vi "Submodule EOL UI.vi"() -> ()   [LabVIEW 2025, in "Submodule EOL.lvlib" / "Submodule EOL.lvclass"]
doc: "Copyright 2017 National Instruments Corporation\n\nLicensed under the Apache License, Version 2.0 (the \"License\"); you may not use this file except in compliance with the License. You may obtain a copy of the License at http://www.apache.org/licenses/LICENSE-2.0\nUnless required by applicable law or agreed to in writing, software distributed under the License is distributed on an \"AS IS\" BASIS, WITHOUT WARRANTIES OR CONDITIONS OF ANY KIND, either express or implied. See the License for the specific language governing permissions and limitations under the License."
uses:
  Submodule EOL.lvclass
  Users/Public/Documents/Sandia National Labs/TSS Plugin/CEF.lvlibp/Node/mainQref.ctl
  Users/Public/Documents/Sandia National Labs/TSS Plugin/CEF.lvlibp/Node/UserEventRef.ctl
  Submodule EOL configuration/Setting.ctl
  Submodule EOL configuration/PLC.ctl
  Users/Public/Documents/Sandia National Labs/TSS Plugin/CEF.lvlibp/Node/NodeRef.ctl
  Users/Public/Documents/Sandia National Labs/TSS Plugin/CEF.lvlibp/Node/CEF_Node.lvclass
  Submodule EOL configuration/Instrumnet.ctl
  Submodule EOL.lvclass/Submodule EOL.ctl
  Submodule EOL configuration/Submodule EOL configuration.lvclass/Submodule EOL configuration.ctl
  <vilib>/Utility/miscctls.llb/LVPositionTypeDef.ctl
  Submodule EOL configuration/Read Setting.vi
  Submodule EOL configuration/Read PLC.vi
  Submodule EOL configuration/Read Instrument.vi
  Submodule EOL configuration/Write Setting.vi
  Submodule EOL configuration/Write PLC.vi
  Submodule EOL configuration/Write Instrument.vi
  Submodule EOL configuration/Submodule EOL configuration.lvclass
panel:
  in  "Instrument":T1
  in  "node ref":T2
  in  "PLC":T3={"PLC Folder Names"=[["Station0_Rx", "OP50A_TesterRxSignals"], ["Station0_Tx", "OP50A_TesterTxSignals"], ["Station1_Rx", "OP50B_TesterRxSignals"], ["Station1_Tx", "OP50B_TesterTxSignals"], ["Station2_Rx", "OP60A_TesterRxSignals"], ["Station2_Tx", "OP60A_TesterTxSignals"], ["Station3_Rx", "OP60B_TesterRxSignals"], ["Station3_Tx", "OP60B_TesterTxSignals"], ["Station4_Rx", "OP70A_TesterRxSignals"], ["Station4_Tx", "OP70A_TesterTxSignals"], ["Station5_Rx", "OP70B_TesterRxSignals"], ["Station5_Tx", "OP70B_TesterTxSignals"]], "PLC URL"="opc.tcp://localhost:49580 ", "Ignition Folder Names"=[["Ignition0_Rx", "[Submodule_EOL]/StaA/TesterRx"], ["Ignition0_Tx", "[Submodule_EOL]/StaA/TesterTx"], ["Ignition1_Rx", "[Submodule_EOL]/StaB/TesterRx"], ["Ignition1_Tx", "[Submodule_EOL]/StaB/TesterTx"], ["Ignition2_Rx", "[Submodule_EOL]/StaC/TesterRx"], ["Ignition2_Tx", "[Submodule_EOL]/StaC/TesterTx"], ["Ignition3_Rx", "[Submodule_EOL]/StaD/TesterRx"], ["Ignition3_Tx", "[Submodule_EOL]/StaD/TesterTx"], ["Ignition4_Rx", "[Submodule_EOL]/StaE/TesterRx"], ["Ignition4_Tx", "[Submodule_EOL]/StaE/TesterTx"], ["Ignition5_Rx", "[Submodule_EOL]/StaF/TesterRx"], ["Ignition5_Tx", "[Submodule_EOL]/StaF/TesterTx"]], "Ignition URL"="opc.tcp://10.64.0.22:62541/discovery", "Test Name"="Battery Submodule EOL"}
  in  "Segmented":enum32{"PLC", "Setting", "Instrument"}(radio)
  in  "Setting":T4={"Local Database"="", "Connect OPC Trial"=0, "Timeout Connect OPC"=0.0, "AbstractUUT Path"="", "PreUUT Path"="", "Test Path"="", "PostUUT Path"="Battery Submodule End of Line"} {"Timeout Connect OPC" format="%#_f"}
  in  "user event":T5
  in  "main queue":T6
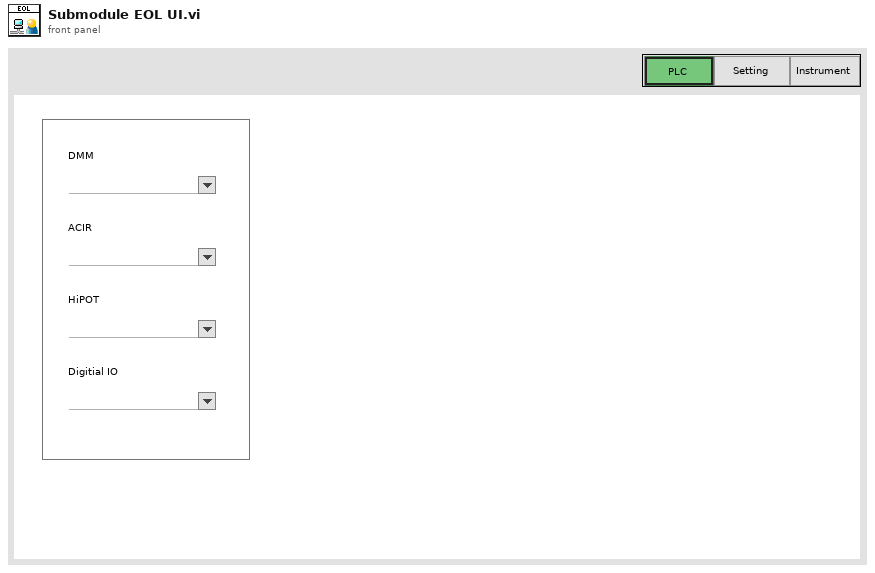
[diagram p1: front panel]
types:
  T1 = typedef "Submodule EOL.lvlib/Submodule EOL configuration.lvclass/Instrumnet.ctl" = cluster{"Digitial IO":string, "HiPOT":string, "ACIR":string, "DMM":string}
  T2 = typedef "CEF.lvlibp/CEF_Node.lvclass/NodeRef.ctl" = refnum<data-value>
  T3 = typedef "Submodule EOL.lvlib/Submodule EOL configuration.lvclass/PLC.ctl" = cluster{"PLC Folder Names":string[][], "PLC URL":string, "Ignition Folder Names":string[][], "Ignition URL":string, "Test Name":string}
  T4 = typedef "Submodule EOL.lvlib/Submodule EOL configuration.lvclass/Setting.ctl" = cluster{"Local Database":string, "Connect OPC Trial":u32, "Timeout Connect OPC":dbl, "AbstractUUT Path":string, "PreUUT Path":string, "Test Path":string, "PostUUT Path":string}
  T5 = typedef "CEF.lvlibp/CEF_Node.lvclass/UserEventRef.ctl" = refnum<user-event>
  T6 = typedef "CEF.lvlibp/CEF_Node.lvclass/mainQref.ctl" = refnum<queue>
  T7 = typedef "LVPositionTypeDef.ctl" = cluster{"Left":i32, "Top":i32}
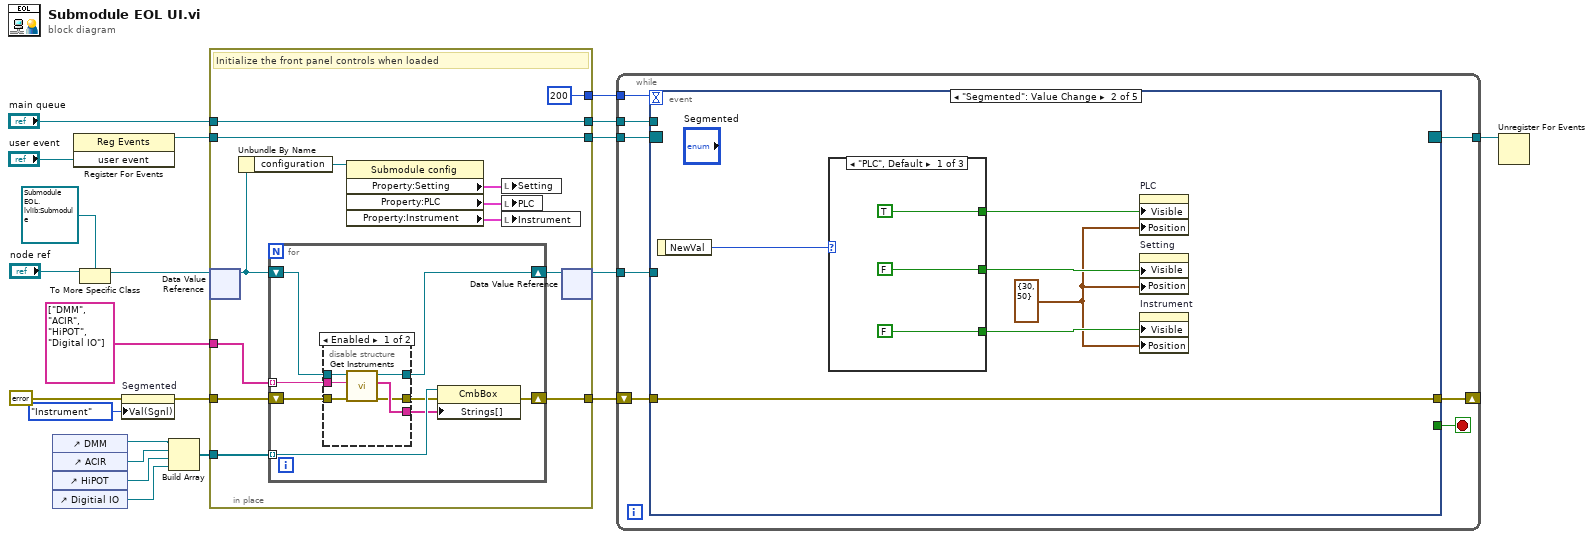
[diagram p0: block diagram]
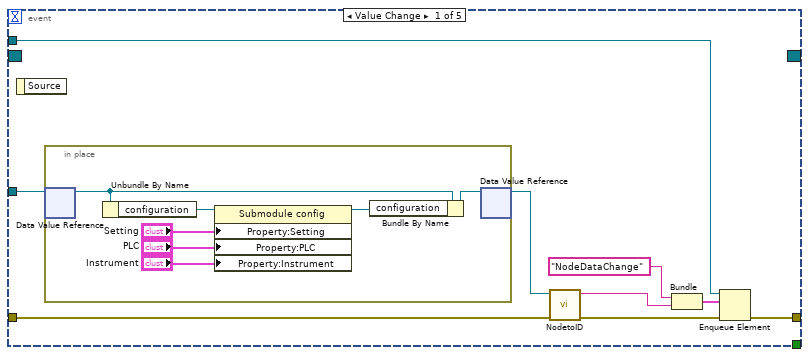
[diagram p3: hidden frame]
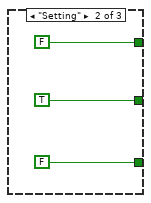
[diagram p4: hidden frame]
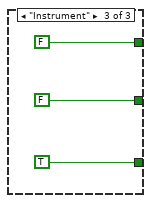
[diagram p5: hidden frame]
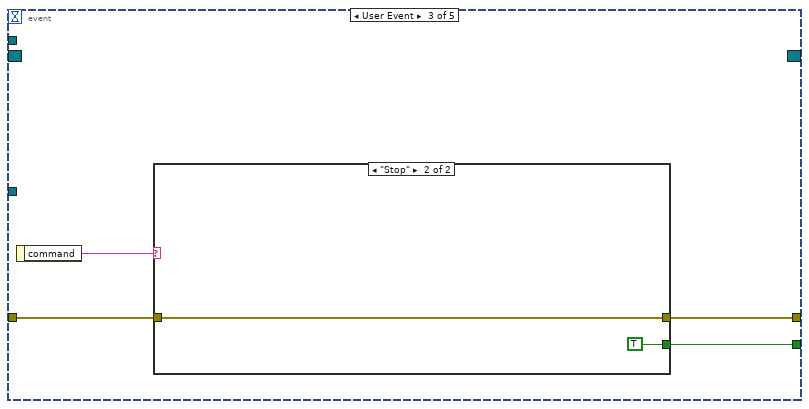
[diagram p6: hidden frame]
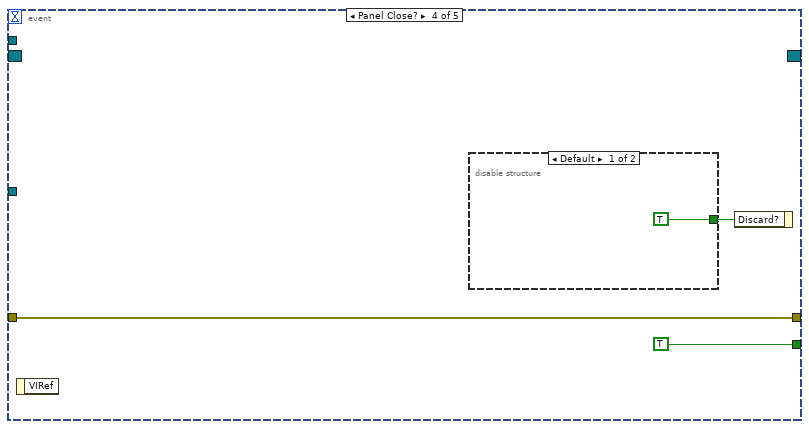
[diagram p8: hidden frame]
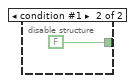
[diagram p9: hidden frame]
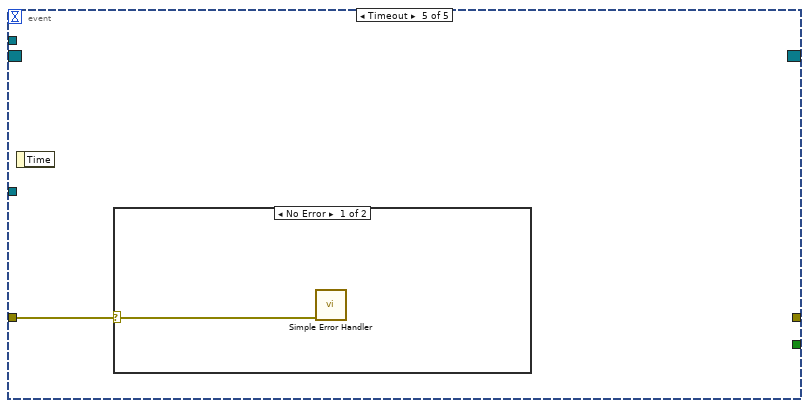
[diagram p10: hidden frame]
diagram:
  n1 = control-ref of="DMM"() -> (w2:refnum<vi>)
  n2 = control-ref of="ACIR"() -> (w17:refnum<vi>)
  n3 = control-ref of="HiPOT"() -> (w18:refnum<vi>)
  n4 = control-ref of="Digitial IO"() -> (w19:refnum<vi>)
  n5 = register-events("user event") -> (reference out=w7:refnum<event-registration>)  [unwired: 2 in, 1 out]
  n6 = To More Specific Class(target class=refnum<data-value> refnum ("data value reference"), reference="node ref") -> (specific class reference=w13:refnum<data-value>)  [unwired: 1 in, 1 out]
  n7 = property on="Segmented" class="RadioBtnsControl (strict)"(error in=errorcluster {"status"=FALSE, "code"=0, "source"=""} ("error out"), "Val(Sgnl)"=enum32{"PLC", "Setting", "Instrument"}."Instrument" ("Value (Signaling)")) -> (error out=w10:errorcluster)  [unwired: 1 in, 1 out]
  n8 = Build Array(w2, w17, w18, w19) -> (w16:refnum<vi>[])
  n9 = in-place {
    in-place-border: string[] ["DMM", "ACIR", "HiPOT", "Digital IO"] -> [w31]
    in-place-border: w16 -> [w33]
    in-place-border: [w28] -> w9
    in-place-border: "main queue" -> [w32]
    in-place-border: [w32] -> w14
    in-place-border: w10 -> [w30]
    in-place-border: [200] -> w11
    in-place-border: w7 -> [w27]
    in-place-border: [w27] -> w6
    # "Initialize the front panel controls when loaded"
    n10 = in-place-dvr #1(w13) -> (w26:refnum<class "Submodule EOL.lvclass">)  [unwired: 1 out]
    n11 = Unbundle By Name(w26) -> ("configuration"=w34:refnum<class "Submodule EOL configuration.lvclass">)
    n12 = for {
      shift-right: [w35] -> w28
      shift-left: w30 -> [w38]
      tunnel: w31 -> [w39] mode=indexing
      tunnel: w33 -> [w42] mode=indexing
      shift-right: [w40] -> w25
      shift-left: w26 -> [w41]
      n13 = disable-structure shown="Enabled" {
        disable-tunnel: w41 -> [w48 w50]
        disable-tunnel: [w47 w50] -> w40
        disable-tunnel: w39 -> [w46 _]
        disable-tunnel: w38 -> [w45 w49]
        disable-tunnel: [w44 _] -> w37
        disable-tunnel: [w43 w49] -> w36
        frame Enabled {
          n14 = call "Get Instruments.vi"("error in"=w45, "Engine"=w46, "Submodule in"=w48) -> ("error out"=w43:errorcluster, "Instruments"=w44:string[], "Submodule out"=w47:refnum<class "Submodule EOL.lvclass">)  [unwired: 5 in, 1 out]
        }
        frame Disabled {
        }
      }
      n15 = property class="CmbBox"(reference=w42, error in=w36, "Strings[]"=w37) -> (error out=w35:errorcluster)  [unwired: 1 out]
    }
    n16 = property class="Submodule config"(reference=w34) -> ("Property:Setting"=w22:T4, "Property:PLC"=w23:T3, "Property:Instrument"=w24:T1)  [unwired: 1 in, 2 out]
    n17 = local write "Setting"(w22) -> ()
    n18 = local write "PLC"(w23) -> ()
    n19 = local write "Instrument"(w24) -> ()
    n20 = in-place-dvr #1(w25) -> (w21:refnum<data-value>)  [unwired: 1 out]
  }
  n21 = while {
    tunnel: w6 -> [w52]
    tunnel: w14 -> [w54]
    tunnel: w21 -> [w56]
    tunnel: [w53] -> w20
    shift-right: [w57] -> _
    shift-left: w9 -> [w58]
    tunnel: w11 -> [w51]
    stop <- w55 stop-if-true
    n22 = event shown="[1] \"Segmented\": Value Change" {
      selector: w52 -> [_ _ _ _ _]
      dyn-events: [_ _ _ _ _] -> w53
      timeout: w51 -> [_ _ _ _ _]
      tunnel: w58 -> [w59 w79 w91 w99 w102]
      tunnel: [w65 w79 w90 w99 _] -> w57
      tunnel: w56 -> [w67 _ _ _ _]
      tunnel: [_ _ w92 TRUE _] -> w55
      tunnel: w54 -> [w63 _ _ _ _]
      event Value Change {
        n23 = event-data() -> ()  [unwired: 2 out]
        n24 = in-place {
          # "Initialize the front panel controls when loaded"
          n25 = in-place-dvr #2(w67) -> (w71:refnum<class "Submodule EOL.lvclass">)  [unwired: 1 out]
          n26 = Unbundle By Name(w71) -> ("configuration"=w72:refnum<class "Submodule EOL configuration.lvclass">)
          n27 = property class="Submodule config"(reference=w72, "Property:Setting"="Setting", "Property:PLC"="PLC", "Property:Instrument"="Instrument") -> (reference out=w73:refnum<class "Submodule EOL configuration.lvclass">)  [unwired: 1 in, 1 out]
          n28 = Bundle By Name(cluster=w71, "configuration"=w73) -> (w74:refnum<class "Submodule EOL.lvclass">)
          n29 = in-place-dvr #2(w74) -> (w64:refnum<data-value>)  [unwired: 1 out]
        }
        n30 = call "NodetoID.vi"("error in"=w59, "node ref"=w64) -> ("error out"=w66:errorcluster, "ID"=w62:string)  [unwired: 8 in]
        n31 = Bundle("Message Name"="NodeDataChange", "ID"=w62) -> (w61:cluster{"Message Name":string, "ID":string})  [unwired: 1 in]
        n32 = Enqueue Element(queue=w63, element=w61, error in (no error)=w66) -> (error out=w65:errorcluster)  [unwired: 1 in, 2 out]
      }
      event "Segmented": Value Change {
        w75 = T7 {"Left"=30, "Top"=50} ("Position")
        n33 = event-data() -> ("NewVal"=w80:enum32{"PLC", "Setting", "Instrument"})  [unwired: 1 out]
        n34 = case shown="\"PLC\", Default" w80 {
          tunnel: [FALSE ("Visible") TRUE ("Visible") FALSE ("Visible")] -> w78
          tunnel: [TRUE ("Visible") FALSE ("Visible") FALSE ("Visible")] -> w76
          tunnel: [FALSE ("Visible") FALSE ("Visible") TRUE ("Visible")] -> w77
          frame "PLC", Default {
          }
          frame "Setting" {
          }
          frame "Instrument" {
          }
        }
        n35 = property on="PLC" class="Clust (strict)"("Visible"=w76, "Position"=w75) -> ()  [unwired: 2 in, 2 out]
        n36 = property on="Setting" class="Clust (strict)"("Visible"=w78, "Position"=w75) -> ()  [unwired: 2 in, 2 out]
        n37 = property on="Instrument" class="Clust (strict)"("Visible"=w77, "Position"=w75) -> ()  [unwired: 2 in, 2 out]
      }
      event User Event {
        n38 = event-data() -> ("command"=w93:string)  [unwired: 1 out]
        n39 = case shown="\"Stop\"" w93 {
          tunnel: [_ TRUE] -> w92
          tunnel: w91 -> [w94 w95]
          tunnel: [w94 w95] -> w90
          frame Default {
          }
          frame "Stop" {
          }
        }
      }
      event Panel Close? {
        n40 = event-data() -> ()  [unwired: 2 out]
        n41 = disable-structure shown="Default" {
          disable-tunnel: [TRUE FALSE] -> w97
          frame condition #0 (active) {
          }
          frame condition #1 {
          }
        }
        n42 = event-data("Discard?"=w97) -> ()  [unwired: 1 in, 1 out]
      }
      event Timeout {
        n43 = event-data() -> ()  [unwired: 2 out]
        n44 = case shown="No Error" w102 {
          selector: w102 -> [w103 _]
          frame No Error {
            n45 = call <vilib>:"Simple Error Handler.vi"("error in (no error)"=w103) -> ()  [unwired: 4 in, 5 out]
          }
          frame Error {
          }
        }
      }
    }
  }
  n46 = Unregister For Events(event registration refnum=w20) -> ()  [unwired: 1 in, 1 out]
